vi "GetAttributes.vi"(0 "ClassReaderNative in":refnum<class "ClassReaderNative.lvclass">, 1 "OnlyGetReference":bool, 5 "error in (no error)":errorcluster) -> (14 "ClassReaderNative out":refnum<class "ClassReaderNative.lvclass">, 15 "ObjectAttributes":T1[](array[typedef])=[{"name"="MyU8", "type"=enum."UINT8", "dimension"=0, "typeName"="", "typePath"=path "", "visibility"=enum."Protected"}, {"name"="MyStrArray", "type"=enum."STRING", "dimension"=1, "typeName"="", "typePath"=path "", "visibility"=enum."Protected"}], 16 "ClassAttributes":T1[](array[typedef])=[{"name"="MyU8", "type"=enum."UINT8", "dimension"=0, "typeName"="", "typePath"=path "", "visibility"=enum."Protected"}, {"name"="MyStrArray", "type"=enum."STRING", "dimension"=1, "typeName"="", "typePath"=path "", "visibility"=enum."Protected"}], 17 "ObjectAttributeReference":refnum<vi>, 18 "ClassAttributeReference":refnum<vi>, 19 "error out":errorcluster)   [LabVIEW 2020, in "ClassReaderNative.lvclass"]
uses:
  ClassReaderNative.lvclass
  Common/CommonVIs/CommonVIs_AttributeInfoType.ctl
  Common/CommonVIs/CommonVIs_AttributeDataType.ctl
  Common/CommonVIs/CommonVIs_VisibilityType.ctl
  ClassReaderNative.lvclass/ClassReaderNative.ctl
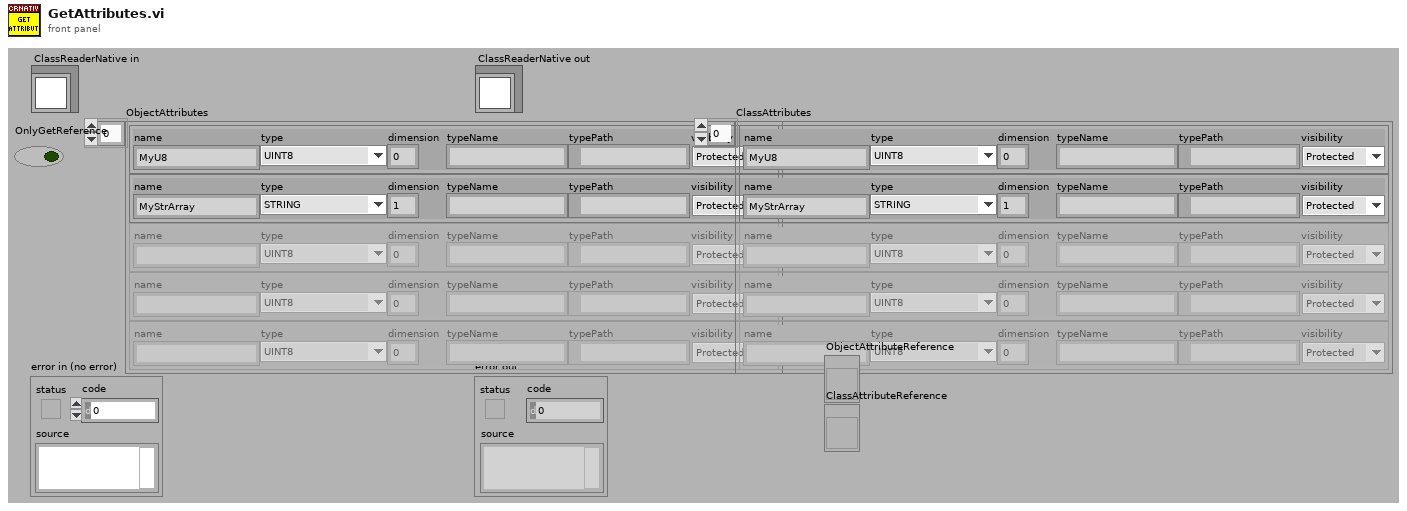
[diagram p1: front panel]
types:
  T1 = typedef "CommonVIs_AttributeInfoType.ctl" = cluster{"name":string, "type":T2, "dimension":i32, "typeName":string, "typePath":path, "visibility":T3}
  T2 = typedef "CommonVIs_AttributeDataType.ctl" = enum16{"UINT8", "INT8", "UINT16", "INT16", "UINT32", "INT32", "UINT64", "INT64", "SGL", "DBL", "EXT", "CSG", "CDB", "CXT", "TimeStamp", "STRING", "PATH", "BOOL", "ENUM", "RefNum", "VIRefNum", "LabVIEW Class", "Cluster", "Variant", "TypeDef", "Waveform", "LabVIEW Object", "Other", "void", "Set", "Map"}
  T3 = typedef "CommonVIs_VisibilityType.ctl" = enum16{"Public", "Private", "Protected"}
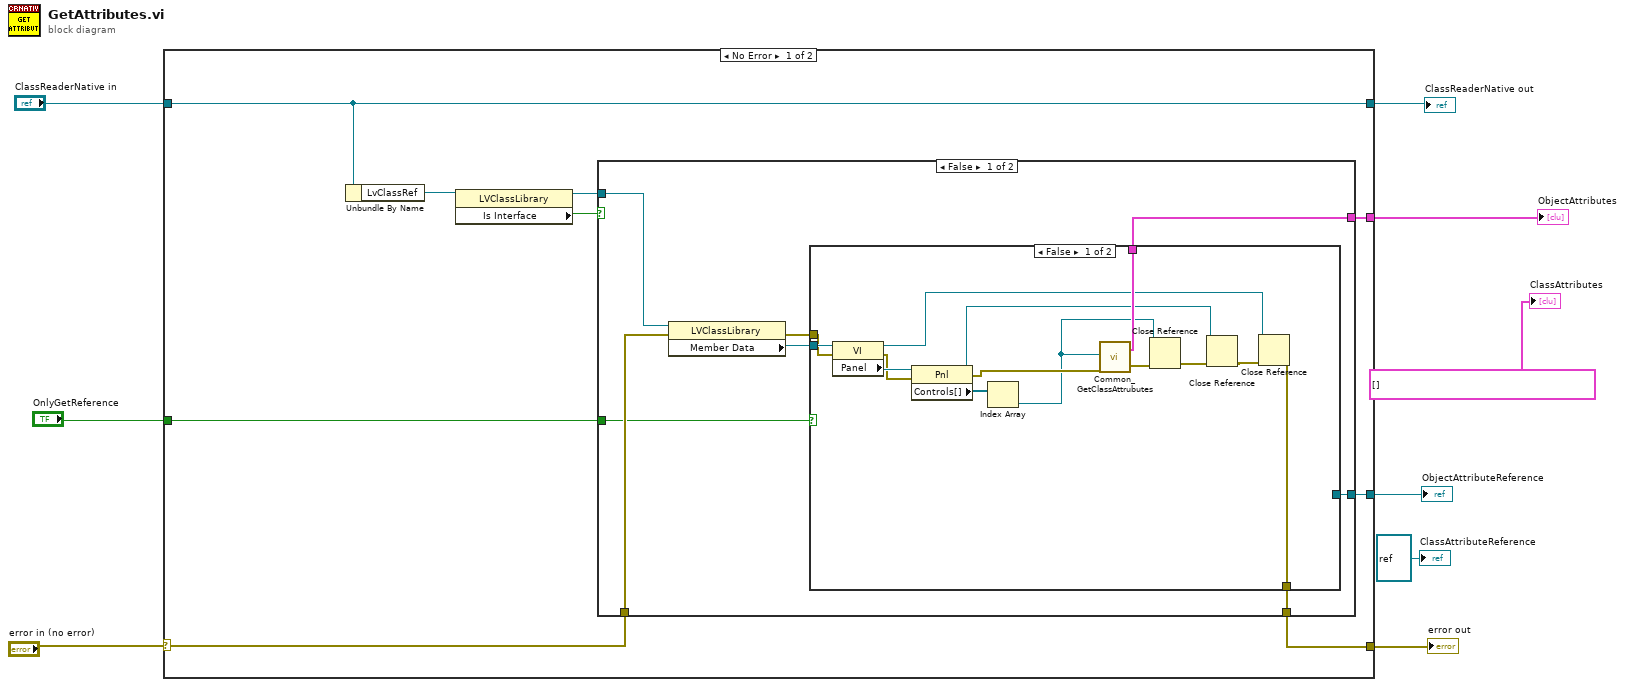
[diagram p0: block diagram]
diagram:
  n1 = case shown="No Error" "error in (no error)" {
    selector: "error in (no error)" -> [w17 w44]
    tunnel: "ClassReaderNative in" -> [w16 w45]
    tunnel: [w16 w45] -> w7
    tunnel: [w15 w44] -> w6
    tunnel: [w18 _] -> w5
    tunnel: "OnlyGetReference" -> [w13 _]
    tunnel: [w14 _] -> w2
    frame No Error {
      n2 = Unbundle By Name(w16) -> ("LvClassRef"=w12:refnum<vi>)
      n3 = property class="LVClassLibrary"(reference=w12) -> (reference out=w11:refnum<vi>, "Is Interface"=w10:bool)  [unwired: 1 in, 1 out]
      n4 = case shown="False" w10 {
        tunnel: [w24 _] -> w18
        tunnel: w17 -> [w23 w43]
        tunnel: [w22 w43] -> w15
        tunnel: [w21 _] -> w14
        tunnel: w13 -> [w20 _]
        tunnel: w11 -> [w19 _]
        frame False {
          n5 = property class="LVClassLibrary"(reference=w19, error in=w23) -> (error out=w25:errorcluster, "Member Data"=w26:refnum<vi>)  [unwired: 1 out]
          n6 = case shown="False" w20 {
            tunnel: w26 -> [w40 w41]
            tunnel: w25 -> [w39 w42]
            tunnel: [w34 _] -> w24
            tunnel: [w27 w42] -> w22
            tunnel: [_ w41] -> w21
            frame False {
              n7 = property class="VI"(reference=w40, error in=w39) -> (reference out=w29:refnum<vi>, error out=w35:errorcluster, "Panel"=w37:refnum<vi>)
              n8 = property class="Pnl"(reference=w37, error in=w35) -> (reference out=w31:refnum<vi>, error out=w36:errorcluster, "Controls[]"=w38:refnum<vi>[])
              n9 = Index Array(array=w38) -> (element=w33:refnum<vi>)  [unwired: 1 in]
              n10 = call "Common_GetClassAttrubutes.vi"("CtlRefnum"=w33, "error in (no error)"=w36) -> ("attributeInfo"=w34:T1[], "error out"=w28:errorcluster)  [unwired: 15 in, 1 out]
              n11 = Close Reference(reference=w33, error in (no error)=w28) -> (error out=w32:errorcluster)
              n12 = Close Reference(reference=w31, error in (no error)=w32) -> (error out=w30:errorcluster)
              n13 = Close Reference(reference=w29, error in (no error)=w30) -> (error out=w27:errorcluster)
            }
            frame True {
            }
          }
        }
        frame True {
        }
      }
    }
    frame Error {
    }
  }
  "ClassReaderNative out" <- w7
  "error out" <- w6
  "ObjectAttributes" <- w5
  "ObjectAttributeReference" <- w2
  "ClassAttributes" <- T1[] [] ("ClassAttributes")
  "ClassAttributeReference" <- refnum<vi> refnum ("ClassAttributeReference")
